vi "navtcpconversion.vi"() -> ()   [LabVIEW 2023]
panel:
  out "length":i32
  out "error out":errorcluster
  out "code":i32
  in  "timeout ms (25000)":i32=25000
  out "GPS Word (U32)":u32
  out "Status":string
  in  "stop":bool
  in  "Timeout (ms)":dbl
  in  "port":u16
  in  "ip address":string
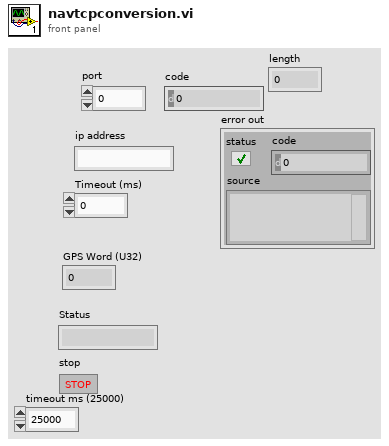
[diagram p1: front panel]
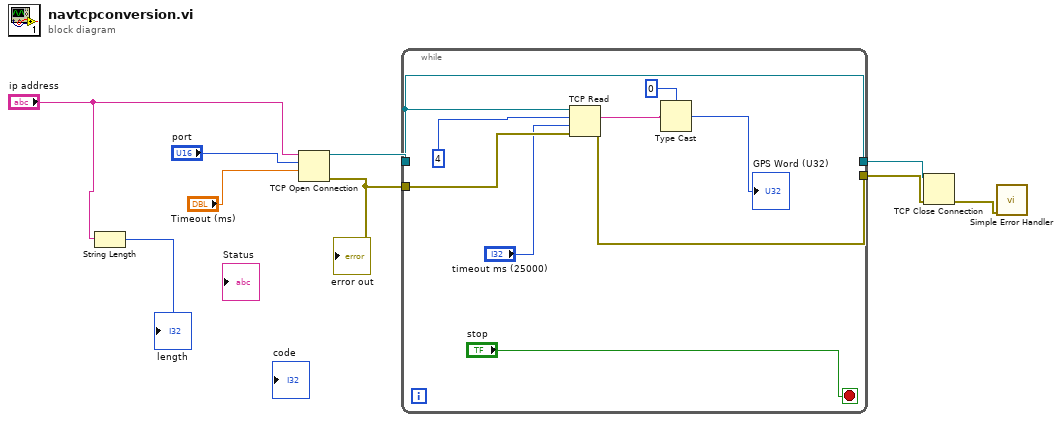
[diagram p0: block diagram]
diagram:
  n1 = String Length(string="ip address") -> (length=→"length":i32)
  n2 = TCP Open Connection(address="ip address", remote port or service name="port", timeout ms (60000)="Timeout (ms)") -> (connection ID=w7:refnum<k5>, error out=w3:errorcluster)  [unwired: 2 in]
  "error out" <- w3
  n3 = while {
    tunnel: w7 -> [w13]
    tunnel: w3 -> [w18]
    tunnel: [w13] -> w6
    tunnel: [w16] -> w5
    stop <- "stop" stop-if-true
    n4 = TCP Read(connection ID=w13, bytes to read=4, error in (no error)=w18, 9:"timeout ms (25000)") -> (data out=w12:string, error out=w16:errorcluster)  [unwired: 1 in, 1 out]
    n5 = Type Cast(type=u32 0, x=w12) -> (*(type *) &x=→"GPS Word (U32)":u32)
  }
  n6 = TCP Close Connection(connection ID=w6, error in (no error)=w5) -> (error out=w4:errorcluster)  [unwired: 1 in, 1 out]
  n7 = call <vilib>:"Simple Error Handler.vi"("error in (no error)"=w4) -> ()  [unwired: 4 in, 5 out]
